vi "Tree.vi"() -> ()   [LabVIEW 2019, in "LV-Data.S3.lvclass"]
uses:
  LV-Data.S3.lvclass
  <vilib>/AWS Toolkit/S3/Bucket/Bucket.lvclass
  LV-Data.AWS CLI/LV-Data.AWS CLI.lvclass
  d02910e8-a69d-41da-b4fe-2bfb8e2a363c.vi
  <vilib>/AWS Toolkit/S3/Storage Class.ctl
  <vilib>/AWS Toolkit/S3/NI_AWS_S3.lvlib
  <vilib>/AWS Toolkit/S3/Owner.ctl
  <vilib>/AWS Toolkit/S3/Object Content.ctl
panel:
  out "get all keys (s)":dbl
  out "list objects (s)":dbl
  out "Current State":string
  out "Active Item:Tag":string
  out "All Tags":string[](array[string])
  in  "OK":bool
  in  "Remote Tree":string(tree)
  out "# objects":i32
  out "Objects":T1[](array[typedef])
  out "populate tree (s)":dbl
  # "LV API: 91512 objects / 80.19 seconds  \nCLI     : 91512 objects / 260.977 seconds"
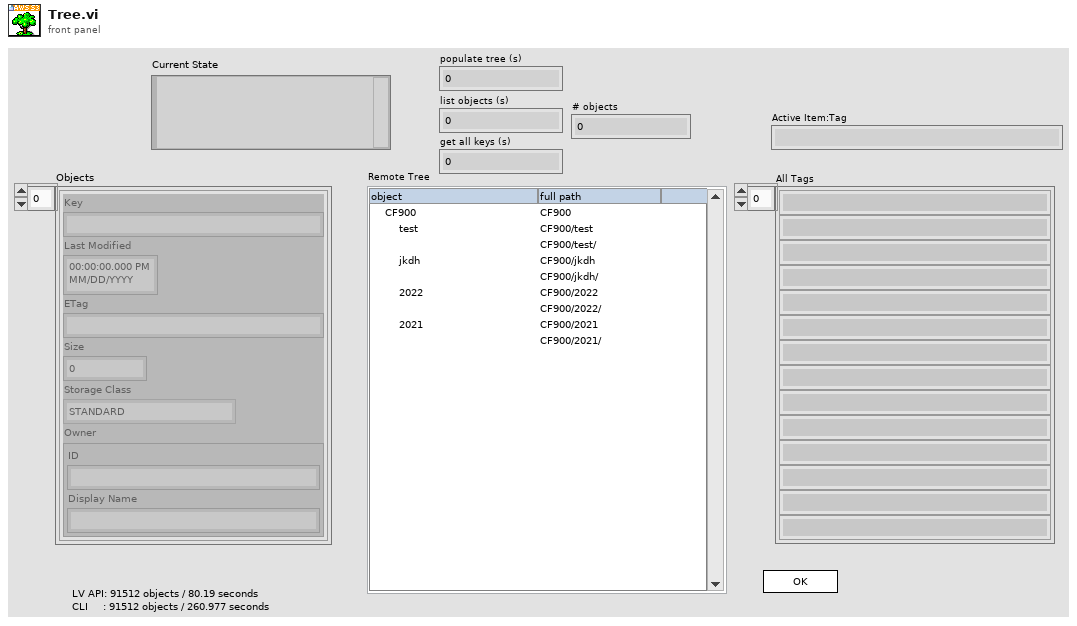
[diagram p1: front panel]
types:
  T1 = typedef "NI_AWS_S3.lvlib/Object Content.ctl" = cluster{"Key":string, "Last Modified":timestamp, "ETag":string, "Size":u64, "Storage Class":T2, "Owner":T3}
  T2 = typedef "NI_AWS_S3.lvlib/Storage Class.ctl" = enum16{"STANDARD", "REDUCED_REDUNDANCY"}
  T3 = typedef "NI_AWS_S3.lvlib/Owner.ctl" = cluster{"ID":string, "Display Name":string}
  T4 = typedef "NI_AWS_Core.lvlib/HTTP Request.lvclass/AWS Credentials.ctl" = cluster{"Access Key":string, "Secret Key":string}
  T5 = enum32{"Invalid", "Standard", "Closed", "Hidden", "Minimized", "Maximized"}
  T6 = enum32{"invalid app kind", "Development System", "Run Time System", "Student Edition", "Embedded LabVIEW", "Evaluation", "Custom"}
  T7 = cluster{"Core":cluster{"Current VI Reference":refnum<vi>, "Close Panel on Exit?":bool}, "Remote Tree":refnum<vi>, "all tags":string[]}
  T8 = cluster{"Current VI Reference":refnum<vi>, "Close Panel on Exit?":bool}
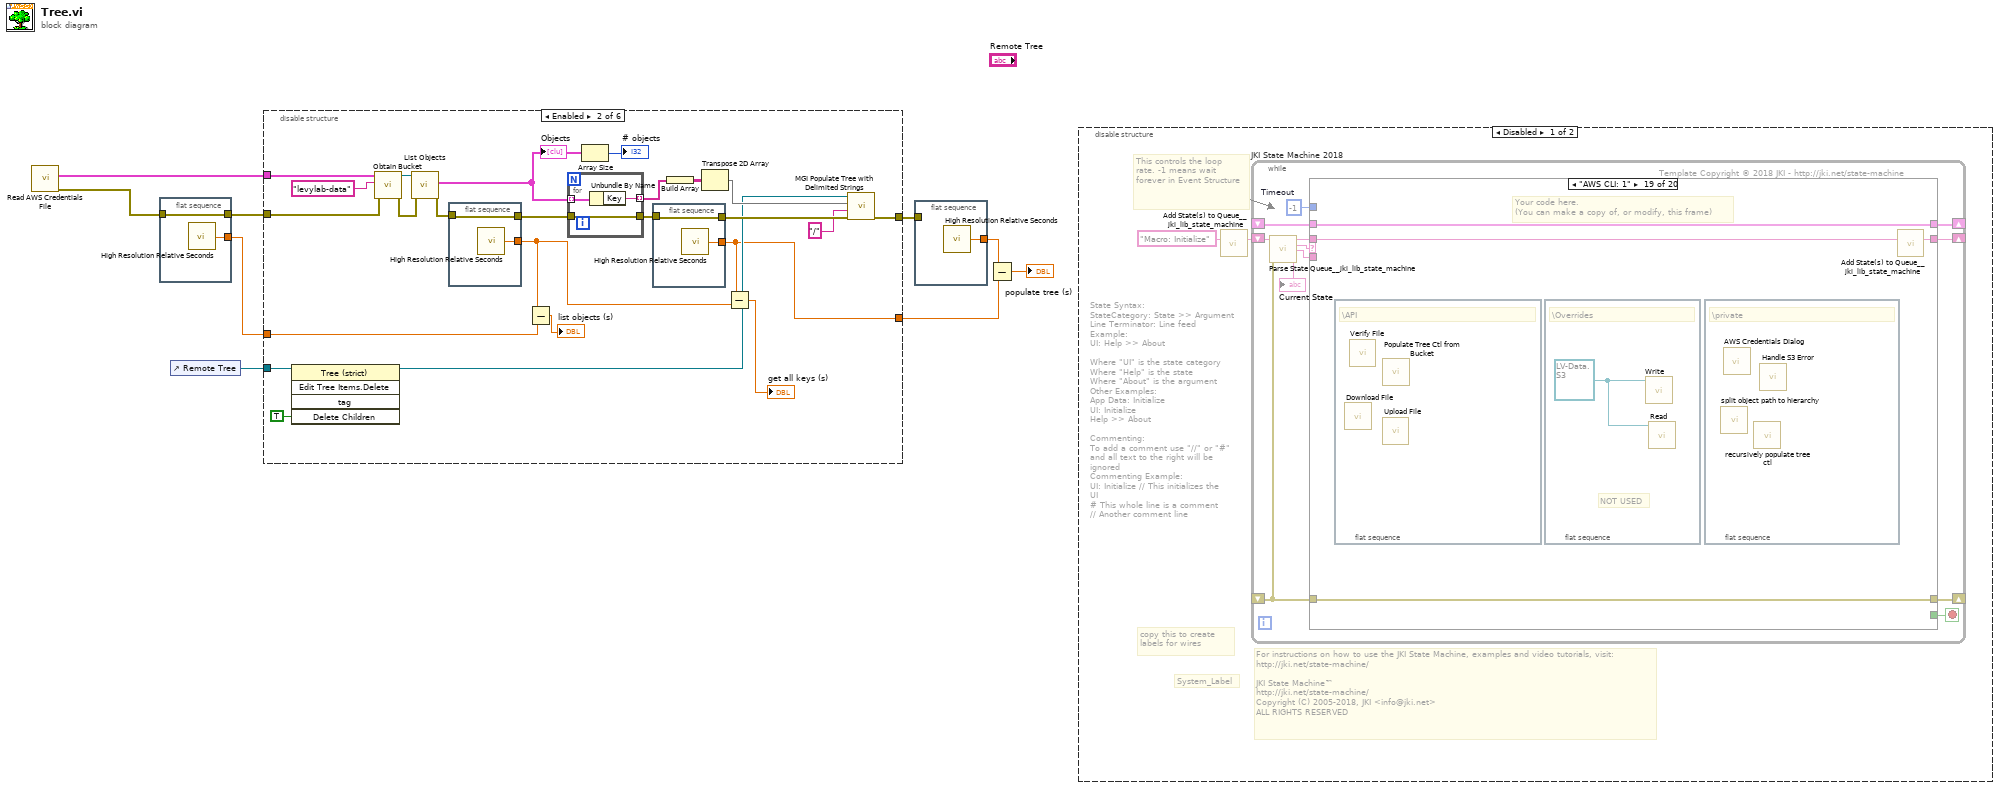
[diagram p0: block diagram]
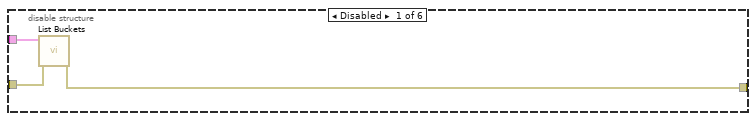
[diagram p2: hidden frame]
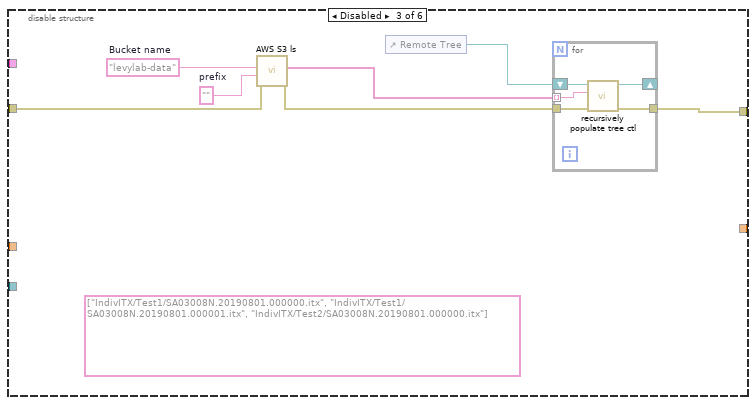
[diagram p3: hidden frame]
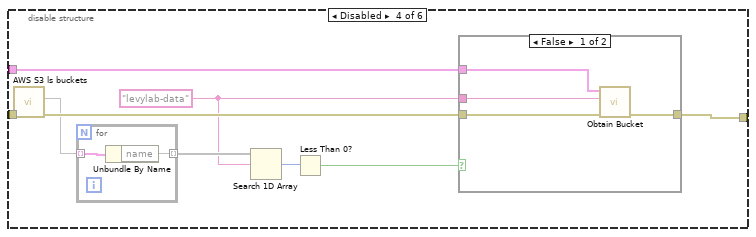
[diagram p4: hidden frame]
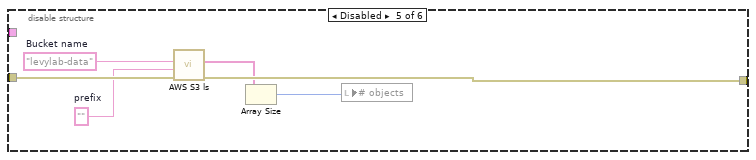
[diagram p6: hidden frame]
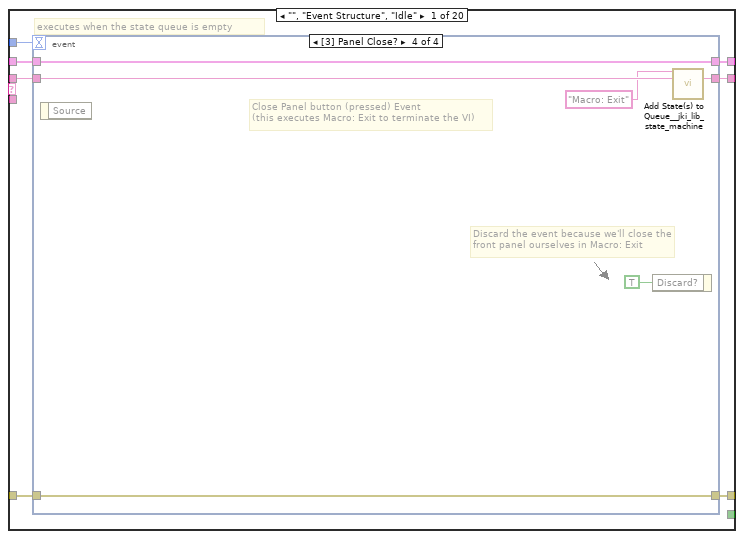
[diagram p8: hidden frame]
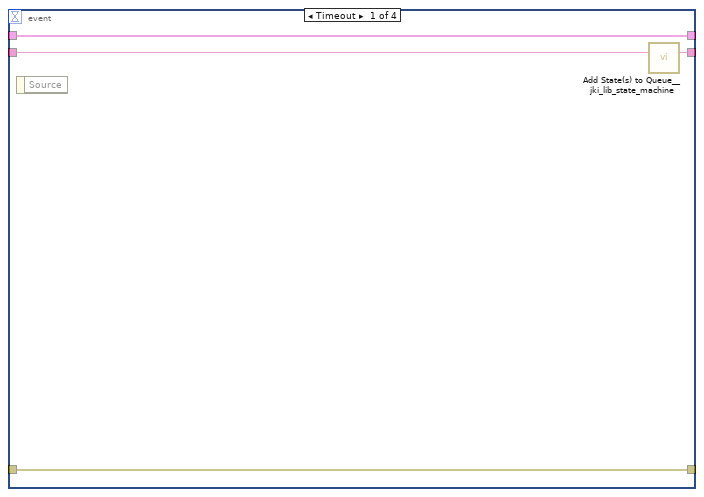
[diagram p9: hidden frame]
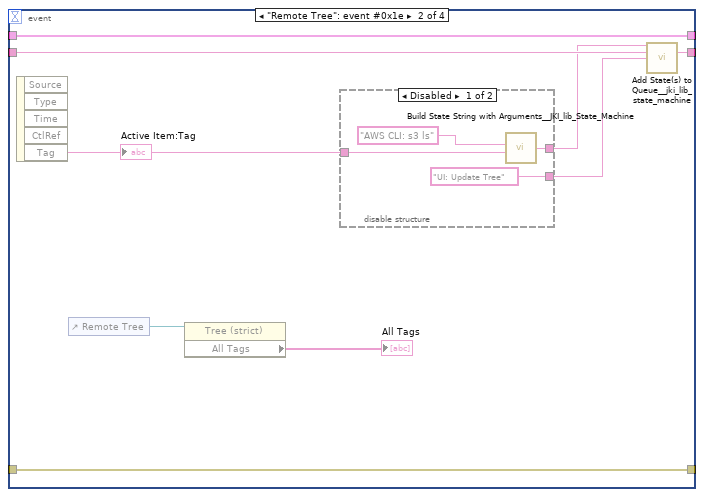
[diagram p10: hidden frame]
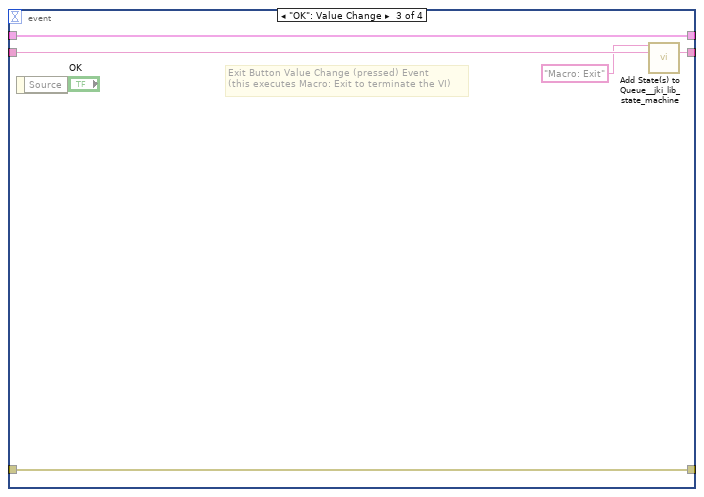
[diagram p12: hidden frame]
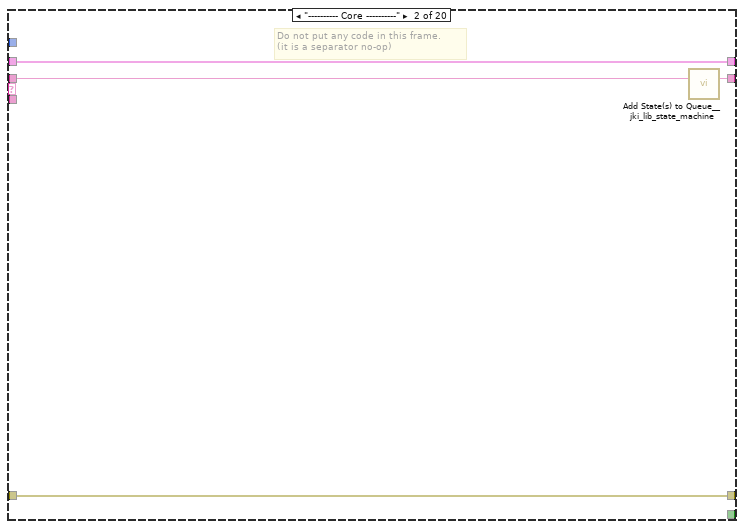
[diagram p13: hidden frame]
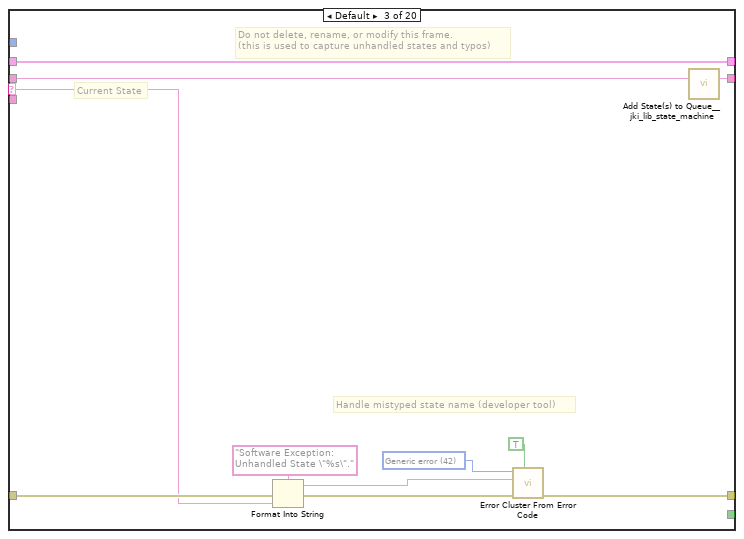
[diagram p14: hidden frame]
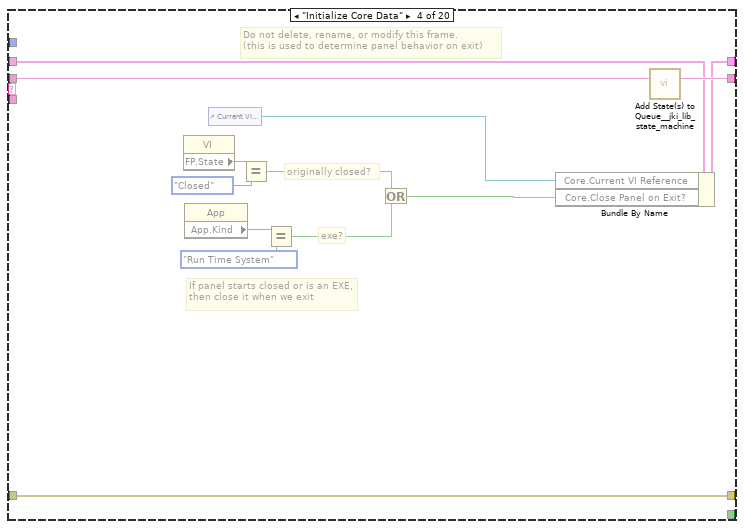
[diagram p15: hidden frame]
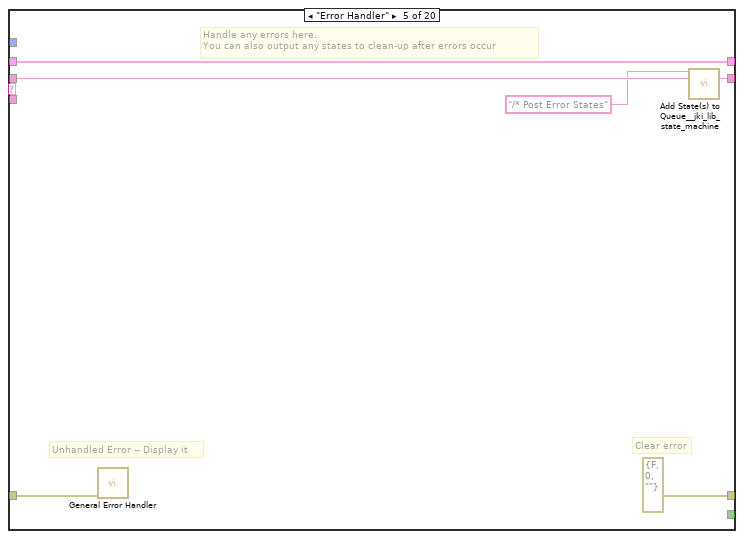
[diagram p16: hidden frame]
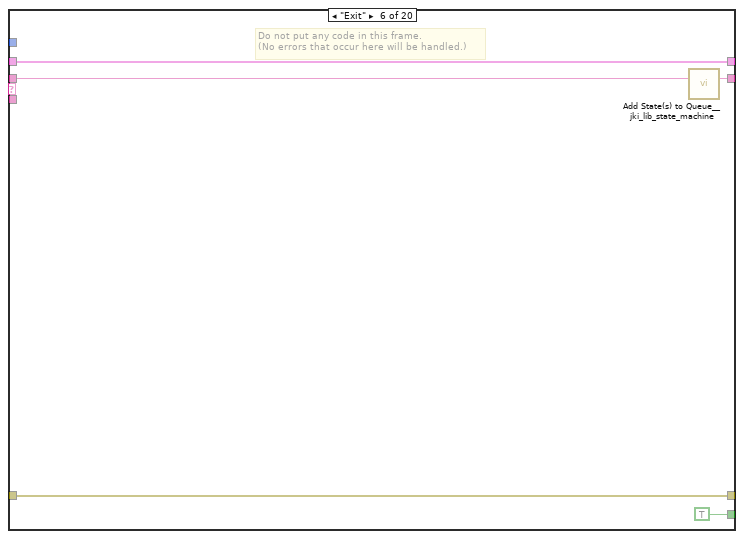
[diagram p17: hidden frame]
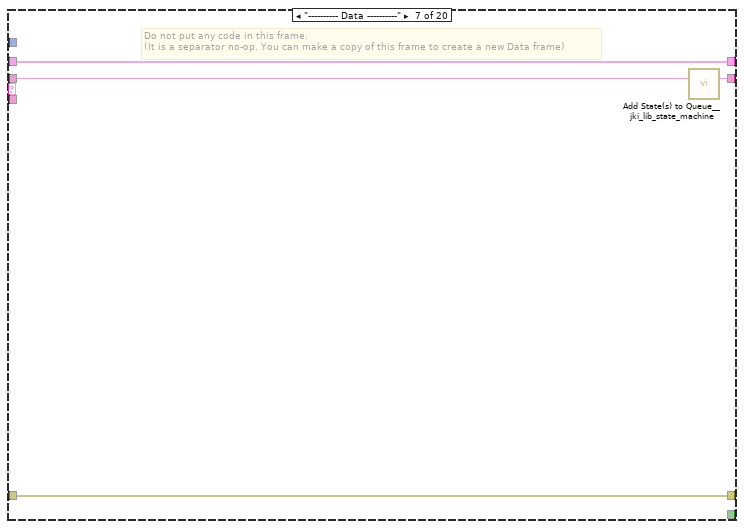
[diagram p18: hidden frame]
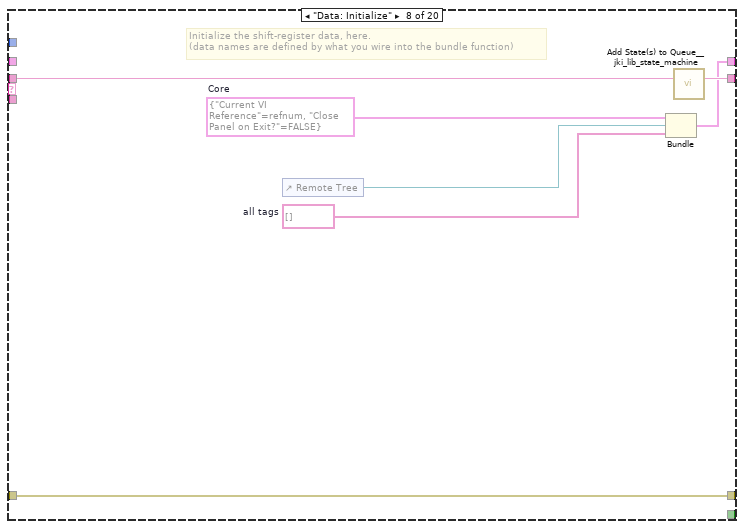
[diagram p19: hidden frame]
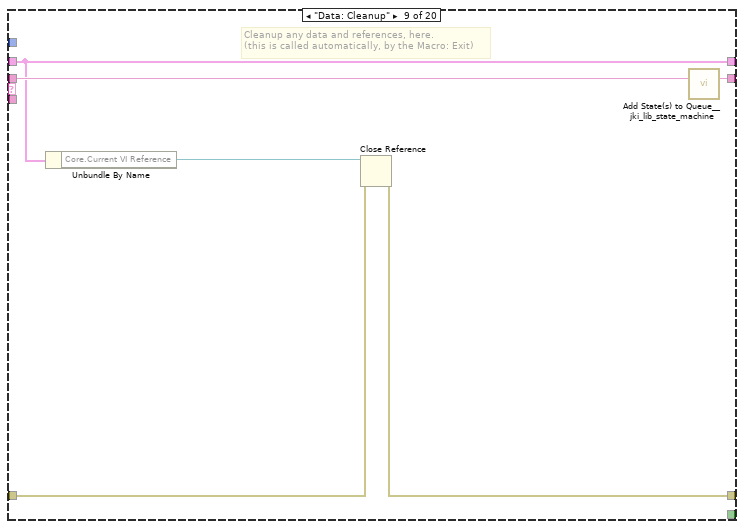
[diagram p20: hidden frame]
diagram:
  n1 = call "Read AWS Credentials File.vi"() -> ("error out"=w7:errorcluster, "AWS Credentials"=w9:T4)  [unwired: 9 in, 1 out]
  n2 = flat-sequence {
    tunnel: [w11] -> w3
    tunnel: w7 -> [w10]
    tunnel: [w10] -> w6
    frame #0 {
      n3 = call <vilib>:"High Resolution Relative Seconds.vi"() -> ("relative seconds"=w11:dbl)
    }
  }
  n4 = control-ref of="Remote Tree"() -> (w2:refnum<vi>)
  n5 = disable-structure shown="Enabled" {
    disable-tunnel: w9 -> [w14 w38 _ w63 _ _]
    disable-tunnel: w6 -> [w13 w37 w47 w66 w79 _]
    disable-tunnel: [w12 w19 w51 w64 w78 _] -> w5
    disable-tunnel: w3 -> [_ w33 _ _ _ _]
    disable-tunnel: w2 -> [_ w30 _ _ _ _]
    disable-tunnel: [_ w18 _ _ _ _] -> w1
    frame Disabled {
      n6 = call <vilib>:"List Buckets.vi"("error in (no error)"=w13, "AWS Credentials"=w14) -> ("error out"=w12:errorcluster)  [unwired: 6 in, 3 out]
    }
    frame Enabled {
      n7 = invoke class="Tree (strict)" method="Edit Tree Items.Delete"(reference=w30, "Delete Children"=TRUE ("Delete Children?")) -> (reference out=w21:refnum<vi>)  [unwired: 3 in, 4 out]
      n8 = call <vilib>:"Obtain Bucket.vi"("error in (no error)"=w37, "Bucket name"="levylab-data", "AWS Credentials"=w38) -> ("error out"=w31:errorcluster, "Bucket"=w35:refnum<class "Bucket.lvclass">)  [unwired: 7 in]
      n9 = call <vilib>:"List Objects.vi"("error in (no error)"=w31, "Bucket in"=w35) -> ("error out"=w32:errorcluster, "Objects"=w28:T1[])  [unwired: 6 in, 2 out]
      "Objects" <- w28
      n10 = flat-sequence {
        tunnel: [w45] -> w20
        tunnel: w32 -> [w44]
        tunnel: [w44] -> w26
        frame #0 {
          n11 = call <vilib>:"High Resolution Relative Seconds.vi"() -> ("relative seconds"=w45:dbl)
        }
      }
      n12 = Subtract(x=w20, y=w33) -> (x-y=→"list objects (s)":dbl)
      n13 = for {
        tunnel: w28 -> [w43] mode=indexing
        tunnel: [w42] -> w27
        tunnel: w26 -> [w42]
        tunnel: [w41] -> w24 mode=indexing
        n14 = Unbundle By Name(w43) -> ("Key"=w41:string)
      }
      n15 = Array Size(array=w28) -> (size(s)=→"# objects":i32)
      n16 = flat-sequence {
        tunnel: [w40] -> w18
        tunnel: w27 -> [w39]
        tunnel: [w39] -> w25
        frame #0 {
          n17 = call <vilib>:"High Resolution Relative Seconds.vi"() -> ("relative seconds"=w40:dbl)
        }
      }
      n18 = Build Array(w24) -> (w23:string[][])
      n19 = Transpose 2D Array(2D array=w23) -> (transposed array=w22:string[][])
      n20 = Subtract(x=w18, y=w20) -> (x-y=→"get all keys (s)":dbl)
      n21 = call <userlib>:"MGI Populate Tree with Delimited Strings.vi"("error in (no error)"=w25, "Delimiter"="/", "Items (Delimited)"=w22, "Tree Control"=w21) -> ("error out"=w19:errorcluster)  [unwired: 5 in, 2 out]
    }
    frame Disabled {
      w49 = ""  # prefix
      w50 = "levylab-data"  # Bucket name
      (unwired) string[] ["IndivITX/Test1/SA03008N.20190801.000000.itx", "IndivITX/Test1/SA03008N.20190801.000001.itx", "IndivITX/Test2/SA03008N.20190801.000000.itx"]
      n22 = call "AWS S3 ls.vi"("error in (no error)"=w47, "prefix"=w49, "bucket"=w50) -> ("error out"=w48:errorcluster, "Array Output"=w46:string[])  [unwired: 6 in, 1 out]
      n23 = control-ref of="Remote Tree"() -> (w52:refnum<vi>)
      n24 = for {
        shift-right: [w56] -> _
        shift-left: w52 -> [w57]
        tunnel: w48 -> [w55]
        tunnel: [w54] -> w51
        tunnel: w46 -> [w53] mode=indexing
        n25 = call "recursively populate tree ctl.vi"("error in (no error)"=w55, "Object path"=w53, "tree ctl ref"=w57) -> ("error out"=w54:errorcluster, "reference out"=w56:refnum<vi>)  [unwired: 7 in]
      }
    }
    frame Disabled {
      w59 = "levylab-data" ("Bucket name")
      n26 = call "AWS S3 ls buckets.vi"("error in (no error)"=w66) -> ("error out"=w65:errorcluster, 2:w62)  [unwired: 8 in, 1 out]
      n27 = for {
        tunnel: w62 -> [w73] mode=indexing
        tunnel: [w72] -> w61 mode=indexing
        n28 = Unbundle By Name(w73) -> ("name"=w72)
      }
      n29 = Search 1D Array(1D array=w61, element=w59) -> (index of element=w60:i32)  [unwired: 1 in]
      n30 = Less Than 0?(x=w60) -> (x < 0?=w58:bool)
      n31 = case shown="False" w58 {
        tunnel: w65 -> [w70 w71]
        tunnel: [w69 w71] -> w64
        tunnel: w63 -> [w68 _]
        tunnel: w59 -> [w67 _]
        frame False {
          n32 = call <vilib>:"Obtain Bucket.vi"("error in (no error)"=w70, "Bucket name"=w67, "AWS Credentials"=w68) -> ("error out"=w69:errorcluster)  [unwired: 7 in, 1 out]
        }
        frame True {
        }
      }
    }
    frame Disabled {
      w76 = ""  # prefix
      w77 = "levylab-data"  # Bucket name
      n33 = call "AWS S3 ls.vi"("error in (no error)"=w79, "prefix"=w76, "bucket"=w77) -> ("error out"=w78:errorcluster, "Array Output"=w75:string[])  [unwired: 6 in, 1 out]
      n34 = Array Size(array=w75) -> (size(s)=w74:i32)
      n35 = local write "# objects"(w74) -> ()
    }
    frame Disabled {
    }
  }
  n36 = flat-sequence {
    tunnel: [w80] -> w8
    tunnel: w5 -> [_]
    frame #0 {
      n37 = call <vilib>:"High Resolution Relative Seconds.vi"() -> ("relative seconds"=w80:dbl)
    }
  }
  n38 = Subtract(x=w8, y=w1) -> (x-y=→"populate tree (s)":dbl)
  n39 = disable-structure shown="Disabled" {
    frame Disabled {
      # "For instructions on how to use the JKI State Machine, examples and video tutorials, visit:\nhttp://jki.net/state-machine/\n\nJKI State Machine™\nhttp://jki.net/state-machine/\nCopyright (C) 2005-2018, JKI <info@jki.net>\nALL RIGHTS RESERVED"
      # "State Syntax:\nStateCategory: State >> Argument\nLine Terminator: Line feed\nExample:\nUI: Help >> About\n\nWhere \"UI\" is the state category\nWhere \"Help\" is the state\nWhere \"About\" is the argument\nOther Examples:\nApp Data: Initialize\nUI: Initialize\nHelp >> About\n\nCommenting:\nTo add a comment use \"//\" or \"#\" and all text to the right will be ignored\nCommenting Example:\nUI: Initialize // This initializes the UI\n# This whole line is a comment\n// Another comment line"
      # "copy this to create labels for wires"
      # "This controls the loop rate. -1 means wait forever in Event Structure"
      # "System_Label"
      n40 = call <vilib>:"Add State(s) to Queue__jki_lib_state_machine.vi"("State(s) in (\"\")"="Macro: Initialize") -> ("States Out"=w82:string)  [unwired: 14 in]
      n41 = while "JKI State Machine 2018" {
        shift-right: [w86] -> _
        shift-left: _ -> [w85]
        shift-right: [w89] -> _
        shift-left: _ -> [w83]
        shift-right: [w88] -> _
        shift-left: w82 -> [w90]
        stop <- w87 stop-if-true
        w84 = -1  # Timeout
        # "Template Copyright © 2018 JKI - http://jki.net/state-machine"
        n42 = call <vilib>:"Parse State Queue__jki_lib_state_machine.vi"("State Queue"=w90, "Error In (no error)"=w83) -> ("Remaining States"=w92:string, "Current State"=w93:string, "Arguments"=w91:string)  [unwired: 11 in]
        "Current State" <- w93
        n43 = case shown="\"AWS CLI: 1\"" w93 {
          selector: w93 -> [_ _ w133 _ _ _ _ _ _ _ _ _ _ _ _ _ _ _ _ _]
          tunnel: w92 -> [w100 w132 w137 w156 w162 w167 w171 w178 w184 w188 w192 w198 w209 w221 w290 w295 w305 w309 w313 w326]
          tunnel: w91 -> [_ _ _ _ _ _ _ _ _ _ _ w193 _ w215 _ _ _ _ _ w323]
          tunnel: w85 -> [w98 w129 w135 w149 w159 w165 w168 _ w179 w185 w190 w196 w207 w217 w287 w292 w302 w306 w310 w319]
          tunnel: [w97 w130 w139 w153 errorcluster {"status"=FALSE, "code"=0, "source"=""} ("error out") w164 w169 w175 w180 w186 w189 w194 w204 w218 w288 w293 w303 w307 w311 w322] -> w89
          tunnel: w83 -> [w96 w130 w138 w153 w158 w164 w169 w175 w181 w186 w189 w195 w203 w219 w288 w293 w303 w307 w311 w321]
          tunnel: [w99 w131 w136 w155 w161 w166 w170 w177 w183 w187 w191 w197 w208 w220 w289 w294 w304 w308 w312 w325] -> w88
          tunnel: [_ _ _ _ _ TRUE _ _ _ _ _ _ _ _ _ _ _ _ _ _] -> w87
          tunnel: [w95 w129 w135 w154 w159 w165 w168 w176 w179 w185 w190 w196 w207 w217 w287 w292 w302 w306 w310 w320] -> w86
          tunnel: w84 -> [w94 _ _ _ _ _ _ _ _ _ _ _ _ _ _ _ _ _ _ _]
          frame "", "Event Structure", "Idle" {
            # "executes when the state queue is empty"
            n44 = event shown="[3] Panel Close?" {
              selector: _ -> [_ _ _ _]
              dyn-events: _ -> [_ _ _ _]
              timeout: w94 -> [_ _ _ _]
              tunnel: w100 -> [w104 w111 w122 w128]
              tunnel: [w103 w112 w121 w127] -> w99
              tunnel: w98 -> [w101 w113 w119 w125]
              tunnel: [w102 w110 w120 w126] -> w97
              tunnel: w96 -> [w102 w110 w120 w126]
              tunnel: [w101 w113 w119 w125] -> w95
              event Timeout {
                n45 = event-data() -> ()  [unwired: 1 in, 1 out]
                n46 = call <vilib>:"Add State(s) to Queue__jki_lib_state_machine.vi"("State(s) in (\"\")"=w104) -> ("States Out"=w103:string)  [unwired: 14 in]
              }
              event "Remote Tree": event #0x1e {
                n47 = event-data() -> ("Tag"=w107:string)  [unwired: 1 in, 4 out]
                "Active Item:Tag" <- w107
                n48 = control-ref of="Remote Tree"() -> (w109:refnum<vi>)
                n49 = property class="Tree (strict)"(reference=w109) -> ("All Tags"=→"All Tags":string[])  [unwired: 1 in, 2 out]
                n50 = disable-structure shown="Disabled" {
                  disable-tunnel: w107 -> [w116 _]
                  disable-tunnel: [w115 _] -> w106
                  disable-tunnel: ["UI: Update Tree" ("State(s) at Back (\"\")") _] -> w105
                  frame Disabled {
                    n51 = call <vilib>:"Build State String with Arguments__JKI_lib_State_Machine.vi"("Arguments (\"\")"=w116, "State"="AWS CLI: s3 ls") -> ("State with Arguments"=w115:string)  [unwired: 4 in]
                  }
                  frame Enabled {
                  }
                }
                n52 = call <vilib>:"Add State(s) to Queue__jki_lib_state_machine.vi"("State(s) in Front (\"\")"=w106, "State(s) in (\"\")"=w111, "State(s) at Back (\"\")"=w105) -> ("States Out"=w112:string)  [unwired: 12 in]
              }
              event "OK": Value Change {
                # "Exit Button Value Change (pressed) Event\n(this executes Macro: Exit to terminate the VI)"
                n53 = event-data() -> ()  [unwired: 1 in, 1 out]
                n54 = call <vilib>:"Add State(s) to Queue__jki_lib_state_machine.vi"("State(s) in Front (\"\")"="Macro: Exit", "State(s) in (\"\")"=w122) -> ("States Out"=w121:string)  [unwired: 13 in]
              }
              event Panel Close? {
                # "Discard the event because we'll close the front panel ourselves in Macro: Exit"
                # "Close Panel button (pressed) Event\n(this executes Macro: Exit to terminate the VI)"
                n55 = event-data() -> ()  [unwired: 1 in, 1 out]
                n56 = event-data("Discard?"=TRUE) -> ()  [unwired: 1 in, 1 out]
                n57 = call <vilib>:"Add State(s) to Queue__jki_lib_state_machine.vi"("State(s) in Front (\"\")"="Macro: Exit", "State(s) in (\"\")"=w128) -> ("States Out"=w127:string)  [unwired: 13 in]
              }
            }
          }
          frame "---------- Core ----------" {
            # "Do not put any code in this frame.\n(it is a separator no-op)"
            n58 = call <vilib>:"Add State(s) to Queue__jki_lib_state_machine.vi"("State(s) in (\"\")"=w132) -> ("States Out"=w131:string)  [unwired: 14 in]
          }
          frame Default {
            w142 = 42 items=["No error", "Argument error", "Memory is full", "Out of zone", "End of file", "File already open", "Generic file I/O error", "File not found", "File permission error", "Disk is full", "Duplicate path", "Too many files open", "System feature not enabled", "Resource file not found", "Cannot add resource", "Resource not found", "Image not found", "Image memory error", "Pen does not exist", "Config type invalid", "Config token not found", "Config parse error", "Config memory error", "Bad external code format", "Bad external code offset", "External code not present", "Null window", "Destroy window error", "Null menu", "Print aborted", "Bad print record", "Print driver error", "Windows error during printing", "Memory error during printing", "Print dialog error", "Generic print error", "Invalid device refnum", "Device not found", "Device parameter error", "Device unit error", "Cannot open device", "Device call aborted", "Generic error", "Cancelled by user", "Object ID too low", "Object ID too high", "Object not in heap", "Unknown heap", "Unknown object (invalid DefProc)", "Unknown object (DefProc not in table)", "Message out of range", "Invalid (null) method", "Unknown message", "Manager call not supported", "Bad address", "Network operation in progress", "Network operation timed out", "Connection is busy", "Network attribute not supported", "Network error", "Address in use", "System out of memory", "Connection aborted", "Connection refused", "Not connected", "Already connected", "Connection closed", "Initialization error (interapplication manager)", "Bad occurrence", "Wait on unbound occurrence handler", "Occurrence queue overflow", "Datalog type conflict", "Unused", "Unrecognized type (interapplication manager)", "Memory corrupt", "Failed to make temporary DLL", "Old CIN version", "Drag socket not found", "Failed to load drop-object", "Failed to register OLE object", "Failed to release OLE object", "Format specifier type mismatch", "Unknown format specifier", "Too few format specifiers", "Too many format specifiers", "Scan failed", "Newer CIN version", "Error converting to variant", "Runtime menu error", "Password tampered", "Variant attribute not found", "Incompatible variant data type", "Event data is not available", "Event Store is not present", "Occurrence is not found", "Event Queue is not created", "Event info is not available", "Refnum passed is NULL", "Error retrieving Class GUID", "Error retrieving CoClass GUID", "Error retrieving TypeLib GUID.", "Bad built application magic bytes.", "Specific driver is different from the specific driver associated with the Logical Name.", "There is no session opened to the class driver.", "Max Error", "MAX - Error with config objects", "MAX - Error loading configuration", "MAX - Group not supported"]
            # "Current State"
            # "Do not delete, rename, or modify this frame.\n(this is used to capture unhandled states and typos)"
            # "Handle mistyped state name (developer tool)"
            n59 = Format Into String(format string="Software Exception: Unhandled State \"%s\"." ("message"), error in=w138, w133) -> (resulting string=w141:string, error out=w140:errorcluster)  [unwired: 1 in]
            n60 = call <vilib>:"Error Cluster From Error Code.vi"("show call chain? (False)"=TRUE, "error in (no error)"=w140, "error message (\"\")"=w141, "error code (0)"=w142) -> ("error out"=w139:errorcluster)  [unwired: 5 in]
            n61 = call <vilib>:"Add State(s) to Queue__jki_lib_state_machine.vi"("State(s) in (\"\")"=w137) -> ("States Out"=w136:string)  [unwired: 14 in]
          }
          frame "Initialize Core Data" {
            # "Do not delete, rename, or modify this frame.\n(this is used to determine panel behavior on exit)"
            # "originally closed?"
            # "exe?"
            # "If panel starts closed or is an EXE, then close it when we exit"
            n62 = property class="VI"() -> ("FP.State"=w146:T5)  [unwired: 2 in, 2 out]
            n63 = property class="App"() -> ("App.Kind"=w152:T6)  [unwired: 2 in, 2 out]
            n64 = control-ref of="Current VI Reference"() -> (w147:refnum<vi>)
            n65 = Equal?(x=w146, y=T5."Closed" ("Front Panel Window:State")) -> (x = y?=w144:bool)
            n66 = Equal?(x=w152, y=T6."Run Time System" ("Application:Kind")) -> (x = y?=w150:bool)
            n67 = Or(x=w144, y=w150) -> (x .or. y?=w148:bool)
            n68 = Bundle By Name(cluster=w149, "Core.Current VI Reference"=w147, "Core.Close Panel on Exit?"=w148) -> (w154:T7)
            n69 = call <vilib>:"Add State(s) to Queue__jki_lib_state_machine.vi"("State(s) in (\"\")"=w156) -> ("States Out"=w155:string)  [unwired: 14 in]
          }
          frame "Error Handler" {
            # "Unhandled Error -- Display it"
            # "Handle any errors here.\nYou can also output any states to clean-up after errors occur"
            # "Clear error"
            n70 = call <vilib>:"General Error Handler.vi"("error in (no error)"=w158) -> ()  [unwired: 10 in, 5 out]
            n71 = call <vilib>:"Add State(s) to Queue__jki_lib_state_machine.vi"("State(s) in Front (\"\")"="/* Post Error States", "State(s) in (\"\")"=w162) -> ("States Out"=w161:string)  [unwired: 13 in]
          }
          frame "Exit" {
            # "Do not put any code in this frame.\n(No errors that occur here will be handled.)"
            n72 = call <vilib>:"Add State(s) to Queue__jki_lib_state_machine.vi"("State(s) in (\"\")"=w167) -> ("States Out"=w166:string)  [unwired: 14 in]
          }
          frame "---------- Data ----------" {
            # "Do not put any code in this frame.\n(It is a separator no-op. You can make a copy of this frame to create a new Data frame)"
            n73 = call <vilib>:"Add State(s) to Queue__jki_lib_state_machine.vi"("State(s) in (\"\")"=w171) -> ("States Out"=w170:string)  [unwired: 14 in]
          }
          frame "Data: Initialize" {
            w173 = T8 {"Current VI Reference"=refnum, "Close Panel on Exit?"=FALSE}  # Core
            w174 = string[] []  # all tags
            # "Initialize the shift-register data, here.\n(data names are defined by what you wire into the bundle function)"
            n74 = control-ref of="Remote Tree"() -> (w172:refnum<vi>)
            n75 = Bundle("Core"=w173, "Remote Tree"=w172, "all tags"=w174) -> (w176:T7)  [unwired: 1 in]
            n76 = call <vilib>:"Add State(s) to Queue__jki_lib_state_machine.vi"("State(s) in (\"\")"=w178) -> ("States Out"=w177:string)  [unwired: 14 in]
          }
          frame "Data: Cleanup" {
            # "Cleanup any data and references, here.\n(this is called automatically, by the Macro: Exit)"
            n77 = Unbundle By Name(w179) -> ("Core.Current VI Reference"=w182:refnum<vi>)
            n78 = Close Reference(reference=w182, error in (no error)=w181) -> (error out=w180:errorcluster)
            n79 = call <vilib>:"Add State(s) to Queue__jki_lib_state_machine.vi"("State(s) in (\"\")"=w184) -> ("States Out"=w183:string)  [unwired: 14 in]
          }
          frame "---------- UI ----------" {
            # "Do not put any code in this frame.\n(It is a separator no-op. You can make a copy of this frame to create a new UI frame)"
            n80 = call <vilib>:"Add State(s) to Queue__jki_lib_state_machine.vi"("State(s) in (\"\")"=w188) -> ("States Out"=w187:string)  [unwired: 14 in]
          }
          frame "UI: Initialize" {
            # "Initialize the User Interface, here.\n(this is called automatically, by the Macro: Init)"
            n81 = call <vilib>:"Add State(s) to Queue__jki_lib_state_machine.vi"("State(s) in (\"\")"=w192) -> ("States Out"=w191:string)  [unwired: 14 in]
          }
          frame "UI: Cursor Set" {
            # "Argument"
            # "Set and Unset Cursor Busy.\n(Usage: \"UI: Cursor Set >> Busy|Idle\")"
            n82 = case shown="\"Idle\", Default" w193 {
              tunnel: w195 -> [w200 w202]
              tunnel: [w199 w201] -> w194
              frame "Idle", Default {
                n83 = call <vilib>:"Unset Busy.vi"("error in (no error)"=w200) -> ("error out"=w199:errorcluster)  [unwired: 10 in]
              }
              frame "Busy" {
                n84 = call <vilib>:"Set Busy.vi"("error in (no error)"=w202) -> ("error out"=w201:errorcluster)  [unwired: 9 in, 1 out]
              }
            }
            n85 = call <vilib>:"Add State(s) to Queue__jki_lib_state_machine.vi"("State(s) in (\"\")"=w198) -> ("States Out"=w197:string)  [unwired: 14 in]
          }
          frame "UI: Update Tree" {
            # "Do not put any code in this frame.\n(It is a separator no-op. You can make a copy of this frame to create a new UI frame)"
            n86 = Unbundle By Name(w207) -> ("Remote Tree"=w206:refnum<vi>, "all tags"=w205:string[])
            n87 = for {
              shift-right: [w213] -> _
              shift-left: w206 -> [w214]
              tunnel: w203 -> [w212]
              tunnel: [w211] -> w204
              tunnel: w205 -> [w210] mode=indexing
              n88 = call "recursively populate tree ctl.vi"("error in (no error)"=w212, "Object path"=w210, "tree ctl ref"=w214) -> ("error out"=w211:errorcluster, "reference out"=w213:refnum<vi>)  [unwired: 7 in]
            }
            n89 = call <vilib>:"Add State(s) to Queue__jki_lib_state_machine.vi"("State(s) in (\"\")"=w209) -> ("States Out"=w208:string)  [unwired: 14 in]
          }
          frame "UI: Front Panel State" {
            # "Argument"
            # "Set Front Panel Open or Closed\n(Usage: \"UI: Front Panel State >> Open|Close\")"
            n90 = Unbundle By Name(w217) -> ("Core.Current VI Reference"=w216:refnum<vi>)
            n91 = case shown="\"Minimize\", \"Minimized\"" w215 {
              tunnel: w219 -> [w227 w242 w253 w266 w279]
              tunnel: [w229 w243 w255 w268 w281] -> w218
              tunnel: w216 -> [w228 w240 w254 w267 w280]
              frame "Open", "Standard", Default {
                w222 = T5."Standard" ("State")
                n92 = property class="VI"(reference=w228, error in=w227) -> (reference out=w225:refnum<vi>, error out=w226:errorcluster, "FP.State"=w224:T5)
                n93 = Not Equal?(x=w224, y=w222) -> (x != y?=w223:bool)
                n94 = case shown="True" w223 {
                  tunnel: [w233 w235] -> w229
                  tunnel: w226 -> [w232 w235]
                  tunnel: w225 -> [w231 _]
                  tunnel: w222 -> [w230 _]
                  frame True {
                    n95 = invoke class="VI" method="FP.Open"(reference=w231, error in=w232, "Activate"=TRUE, "State"=w230) -> (error out=w233:errorcluster)  [unwired: 1 in, 4 out]
                  }
                  frame False {
                  }
                }
              }
              frame "Close", "Closed" {
                n96 = property class="VI"(reference=w240, error in=w242) -> (reference out=w239:refnum<vi>, error out=w241:errorcluster, "FP.State"=w237:T5)
                n97 = Not Equal?(x=w237, y=T5."Closed" ("Front Panel Window:State")) -> (x != y?=w236:bool)
                n98 = case shown="True" w236 {
                  tunnel: [w244 w247] -> w243
                  tunnel: w241 -> [w244 w246]
                  tunnel: w239 -> [_ w245]
                  frame False {
                  }
                  frame True {
                    n99 = invoke class="VI" method="FP.Close"(reference=w245, error in=w246) -> (error out=w247:errorcluster)  [unwired: 1 in, 2 out]
                  }
                }
              }
              frame "Hidden", "Hide" {
                w248 = T5."Hidden" ("State")
                n100 = property class="VI"(reference=w254, error in=w253) -> (reference out=w251:refnum<vi>, error out=w252:errorcluster, "FP.State"=w250:T5)
                n101 = Not Equal?(x=w250, y=w248) -> (x != y?=w249:bool)
                n102 = case shown="True" w249 {
                  tunnel: [w259 w260] -> w255
                  tunnel: w252 -> [w258 w260]
                  tunnel: w251 -> [w257 _]
                  tunnel: w248 -> [w256 _]
                  frame True {
                    n103 = invoke class="VI" method="FP.Open"(reference=w257, error in=w258, "State"=w256) -> (error out=w259:errorcluster)  [unwired: 2 in, 4 out]
                  }
                  frame False {
                  }
                }
              }
              frame "Minimize", "Minimized" {
                w261 = T5."Minimized" ("State")
                n104 = property class="VI"(reference=w267, error in=w266) -> (reference out=w264:refnum<vi>, error out=w265:errorcluster, "FP.State"=w263:T5)
                n105 = Not Equal?(x=w263, y=w261) -> (x != y?=w262:bool)
                n106 = case shown="True" w262 {
                  tunnel: [w272 w273] -> w268
                  tunnel: w265 -> [w271 w273]
                  tunnel: w264 -> [w270 _]
                  tunnel: w261 -> [w269 _]
                  frame True {
                    n107 = invoke class="VI" method="FP.Open"(reference=w270, error in=w271, "State"=w269) -> (error out=w272:errorcluster)  [unwired: 2 in, 4 out]
                  }
                  frame False {
                  }
                }
              }
              frame "Maximize", "Maximized" {
                w274 = T5."Maximized" ("State")
                n108 = property class="VI"(reference=w280, error in=w279) -> (reference out=w277:refnum<vi>, error out=w278:errorcluster, "FP.State"=w276:T5)
                n109 = Not Equal?(x=w276, y=w274) -> (x != y?=w275:bool)
                n110 = case shown="True" w275 {
                  tunnel: [w285 w286] -> w281
                  tunnel: w278 -> [w284 w286]
                  tunnel: w277 -> [w283 _]
                  tunnel: w274 -> [w282 _]
                  frame True {
                    n111 = invoke class="VI" method="FP.Open"(reference=w283, error in=w284, "State"=w282) -> (error out=w285:errorcluster)  [unwired: 2 in, 4 out]
                  }
                  frame False {
                  }
                }
              }
            }
            n112 = call <vilib>:"Add State(s) to Queue__jki_lib_state_machine.vi"("State(s) in (\"\")"=w221) -> ("States Out"=w220:string)  [unwired: 14 in]
          }
          frame "---------- Macro ----------" {
            # "Do not put any code in this frame.\n(It is a separator no-op. You can make a copy of this frame to create a new Macro frame)"
            n113 = call <vilib>:"Add State(s) to Queue__jki_lib_state_machine.vi"("State(s) in (\"\")"=w290) -> ("States Out"=w289:string)  [unwired: 14 in]
          }
          frame "Macro: Initialize" {
            w291 = "Data: Initialize\nInitialize Core Data\nUI: Initialize\nUI: Front Panel State >> Open\nAWS CLI: s3 ls >> CF900/\nUI: Update Tree"  # Data: Initialize Initialize Core Data UI: Initialize UI: Front Panel State >> Open AWS CLI: s3 ls >> CF900/ UI: Update Tree
            # "Initialization Macro\n(This is called once, when the VI starts)"
            n114 = call <vilib>:"Add State(s) to Queue__jki_lib_state_machine.vi"("State(s) in Front (\"\")"=w291, "State(s) in (\"\")"=w295) -> ("States Out"=w294:string)  [unwired: 13 in]
          }
          frame "Macro: Exit" {
            # "Exit Macro\n(This is called once, when the VI exits)"
            n115 = Unbundle By Name(w302) -> ("Core.Close Panel on Exit?"=w301:bool)
            n116 = Select(t="UI: Front Panel State >> Close", s=w301, f="") -> (s? t:f=w298:string)
            n117 = call <vilib>:"Add State(s) to Queue__jki_lib_state_machine.vi"("State(s) in (\"\")"=w298, "State(s) at Back (\"\")"="Data: Cleanup\nExit") -> ("States Out"=w296:string)  [unwired: 13 in]
            n118 = call <vilib>:"Add State(s) to Queue__jki_lib_state_machine.vi"("State(s) in Front (\"\")"=w296, "State(s) in (\"\")"=w305) -> ("States Out"=w304:string)  [unwired: 13 in]
          }
          frame "---------- AWS CLI ----------" {
            # "Template Separator\n(You can make a copy of, or modify, this frame)"
            n119 = call <vilib>:"Add State(s) to Queue__jki_lib_state_machine.vi"("State(s) in (\"\")"=w309) -> ("States Out"=w308:string)  [unwired: 14 in]
          }
          frame "AWS CLI: 1" {
            # "Your code here.\n(You can make a copy of, or modify, this frame)"
            n120 = flat-sequence {
              frame #0 {
                # "\\API"
                n121 = call "Download File.vi"() -> ()  [unwired: 9 in, 3 out]
                n122 = call "Verify File.vi"() -> ()  [unwired: 9 in, 3 out]
                n123 = call "Upload File.vi"() -> ()  [unwired: 10 in, 2 out]
                n124 = call "Populate Tree Ctl from Bucket.vi"() -> ()  [unwired: 7 in, 5 out]
              }
            }
            n125 = flat-sequence {
              frame #0 {
                w314 = refnum<class "LV-Data.S3.lvclass"> refnum ("Data.S3")
                # "NOT USED"
                # "\\Overrides"
                n126 = call-dynamic "Write.vi"("Data.S3"=w314) -> ()  [unwired: 8 in, 3 out]
                n127 = call-dynamic "Read.vi"("Data.S3"=w314) -> ()  [unwired: 6 in, 5 out]
              }
            }
            n128 = flat-sequence {
              frame #0 {
                # "\\private"
                n129 = call "split object path to hierarchy.vi"() -> ()  [unwired: 8 in, 4 out]
                n130 = call "AWS Credentials Dialog.vi"() -> ()  [unwired: 9 in, 3 out]
                n131 = call "recursively populate tree ctl.vi"() -> ()  [unwired: 10 in, 2 out]
                n132 = call "Handle S3 Error.vi"() -> ()  [unwired: 9 in, 3 out]
              }
            }
            n133 = call <vilib>:"Add State(s) to Queue__jki_lib_state_machine.vi"("State(s) in (\"\")"=w313) -> ("States Out"=w312:string)  [unwired: 14 in]
          }
          frame "AWS CLI: s3 ls" {
            w324 = "levylab-data"  # Bucket name
            # "Your code here.\n(You can make a copy of, or modify, this frame)"
            n134 = Unbundle By Name(w319) -> ("all tags"=w315:string[])
            n135 = call "AWS S3 ls.vi"("error in (no error)"=w321, "prefix"=w323, "bucket"=w324) -> ("error out"=w322:errorcluster, "Array Output"=w316:string[])  [unwired: 6 in, 1 out]
            n136 = Empty Array?(array=w315) -> (empty?=w318:bool)
            n137 = case shown="True" w318 {
              tunnel: [w327 w331] -> w317
              tunnel: w316 -> [w330 w331]
              tunnel: w315 -> [w329 _]
              frame False {
                n138 = Build Array (concatenate)(w329, w330) -> (w328:string[])
                n139 = call "Remove Duplicates From 1D Array.vim"("array"=w328) -> ("array with duplicates removed"=w327:string[])  [unwired: 10 in]
              }
              frame True {
              }
            }
            n140 = Bundle By Name(cluster=w319, "all tags"=w317) -> (w320:T7)
            n141 = call <vilib>:"Add State(s) to Queue__jki_lib_state_machine.vi"("State(s) in (\"\")"=w326) -> ("States Out"=w325:string)  [unwired: 14 in]
          }
        }
      }
    }
    frame Enabled {
    }
  }
